vi "UI_Game_Layout.vi"(11 "error in":errorcluster) -> (4 "Specs":T1(array[cluster]), 15 "error out":errorcluster)   [LabVIEW 2026]
doc: "게임 화면 버튼 배치표. Group 5: 0=무르기, 1=새 게임, 2=설정."
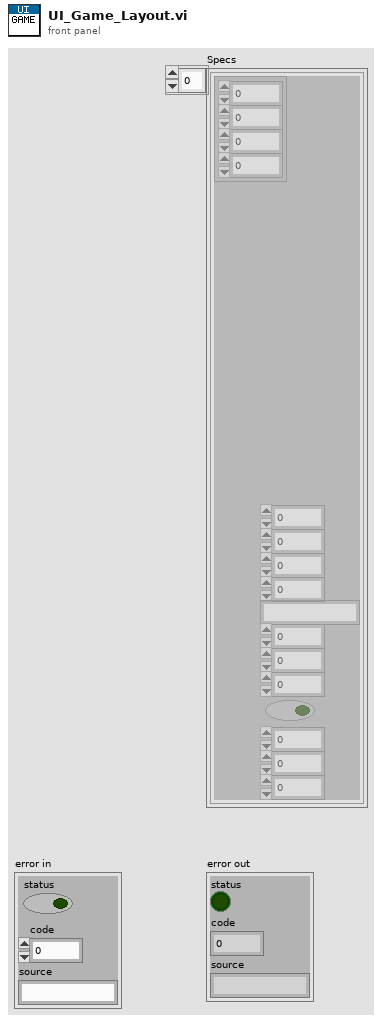
[diagram p1: front panel]
types:
  T1 = cluster{"Rect":cluster{"left":i16, "top":i16, "right":i16, "bottom":i16}, "Fill":u32, "Fill Sel":u32, "Border":u32, "Border Sel":u32, "Text":string, "Text Color":u32, "Text Sel":u32, "Size":i16, "Bold":bool, "Group":i32, "Value":i32, "Radius":i16}[]
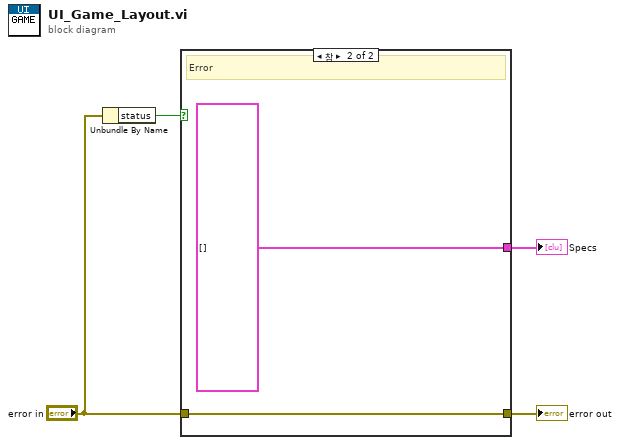
[diagram p0: block diagram]
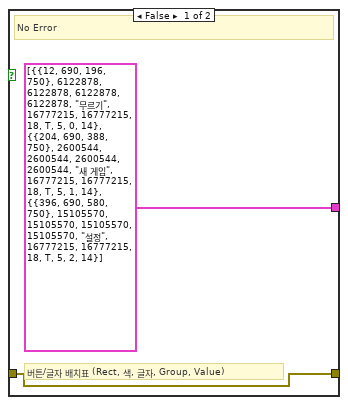
[diagram p2: hidden frame]
diagram:
  n1 = Unbundle By Name("error in") -> ("status"=w2:bool)
  n2 = case shown="참" w2 {
    tunnel: "error in" -> [w5 w7]
    tunnel: [T1 [{"Rect"={"left"=12, "top"=690, "right"=196, "bottom"=750}, "Fill"=6122878, "Fill Sel"=6122878, "Border"=6122878, "Border Sel"=6122878, "Text"="무르기", "Text Color"=16777215, "Text Sel"=16777215, "Size"=18, "Bold"=TRUE, "Group"=5, "Value"=0, "Radius"=14}, {"Rect"={"left"=204, "top"=690, "right"=388, "bottom"=750}, "Fill"=2600544, "Fill Sel"=2600544, "Border"=2600544, "Border Sel"=2600544, "Text"="새 게임", "Text Color"=16777215, "Text Sel"=16777215, "Size"=18, "Bold"=TRUE, "Group"=5, "Value"=1, "Radius"=14}, {"Rect"={"left"=396, "top"=690, "right"=580, "bottom"=750}, "Fill"=15105570, "Fill Sel"=15105570, "Border"=15105570, "Border Sel"=15105570, "Text"="설정", "Text Color"=16777215, "Text Sel"=16777215, "Size"=18, "Bold"=TRUE, "Group"=5, "Value"=2, "Radius"=14}] ("Layout") T1 []] -> w3
    tunnel: [w5 w7] -> w4
    frame False {
      # "버튼/글자 배치표 (Rect, 색, 글자, Group, Value)"
      # "No Error"
    }
    frame True {
      # "Error"
    }
  }
  "Specs" <- w3
  "error out" <- w4
